vi "SDO_DRIVE_MODULE_OPEN.vi"(3 "Module Index":i32, 4 "RadiansPerCount":dbl=1.0, 5 "Drive PWM Channel":T2, 6 "DistancePerCount":dbl=1.0, 7 "Swerve PWM Channel":T2, 8 "Swerve B Channel":T1, 9 "Swerver A Channel":T1, 10 "Drive B Channel":T1, 11 "Drive A channel":T1) -> ()   [LabVIEW 2019]
uses:
  <vilib>/Rock Robotics/SystemInterfaces/DIO/FPGA_DIOChannel.ctl
  <vilib>/Rock Robotics/SystemInterfaces/DIO/FPGA_DIOPWMChannel.ctl
  <vilib>/Rock Robotics/WPI/MotorControl/WPI_MotorControlType.ctl
  <vilib>/Rock Robotics/WPI/PWM/WPI_PWMDeadband.ctl
  <vilib>/Rock Robotics/WPI/MotorControl/WPI_MotorControlDeviceRef.ctl
  <vilib>/Rock Robotics/SystemInterfaces/Encoder/FPGA_EncoderIdx.ctl
  <vilib>/Rock Robotics/SystemInterfaces/Counter/FPGA_CounterCtrSystemIndex.ctl
  <vilib>/Rock Robotics/WPI/Encoder/WPI_EncoderType.ctl
  <vilib>/Rock Robotics/WPI/Encoder/WPI_EncoderDevRef.ctl
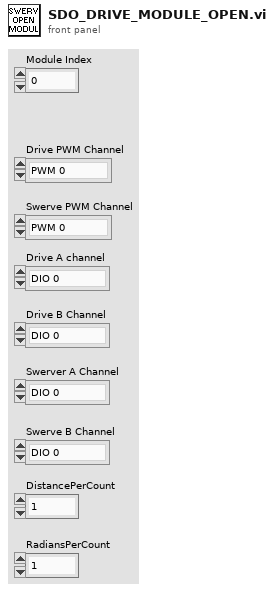
[diagram p1: front panel]
types:
  T1 = typedef "FPGA_DIOChannel.ctl" = enum8{"DIO 0", "DIO 1", "DIO 2", "DIO 3", "DIO 4", "DIO 5", "DIO 6", "DIO 7", "DIO 8", "DIO 9", "DIO MXP 0", "DIO MXP 1", "DIO MXP 2", "DIO MXP 3", "DIO MXP 4", "DIO MXP 5", "DIO MXP 6", "DIO MXP 7", "DIO MXP 8", "DIO MXP 9", "DIO MXP 10", "DIO MXP 11", "DIO MXP 12", "DIO MXP 13", "DIO MXP 14", "DIO MXP 15", "SPI Port CS1", "SPI Port CS2", "SPI Port CS3", "SPI Port MISO", "SPI Port MOSI", "Invalid"}
  T2 = typedef "FPGA_DIOPWMChannel.ctl" = enum8{"PWM 0", "PWM 1", "PWM 2", "PWM 3", "PWM 4", "PWM 5", "PWM 6", "PWM 7", "PWM 8", "PWM 9", "PWM MXP 0", "PWM MXP 1", "PWM MXP 2", "PWM MXP 3", "PWM MXP 4", "PWM MXP 5", "PWM MXP 6", "PWM MXP 7", "PWM MXP 8", "PWM MXP 9", "Invalid"}
  T3 = typedef "WPI_EncoderDevRef.ctl" = cluster{"DevStatus":errorcluster, "EncoderIndex":T4, "CounterIndex":T5, "DistancePerCount":dbl, "Decoding Type":T6}
  T4 = typedef "FPGA_EncoderIdx.ctl" = enum8{"Enc 0", "Enc 1", "Enc 2", "Enc 3", "Enc 4", "Enc 5", "Enc 6", "Enc 7", "Invalid"}
  T5 = typedef "FPGA_CounterCtrSystemIndex.ctl" = enum8{"Ctr 0", "Ctr 1", "Ctr 2", "Ctr 3", "Ctr 4", "Ctr 5", "Ctr 6", "Ctr 7", "Invalid"}
  T6 = typedef "WPI_EncoderType.ctl" = enum16{"1x", "2x", "4x"}
  T7 = typedef "WPI_MotorControlDeviceRef.ctl" = cluster{"DeviceStatus":errorcluster, "Type":T8, "PWM":cluster{"PWM Channel":T2, "DeadBand":T9}, "CAN":cluster{"Device Number":u8, "SetOutput VI Ref":variant, "GetOutput VI Ref":variant, "Enable VI Ref":variant, "Disable VI Ref":variant, "Data":variant}, "Invert":bool, "DIO PWM":cluster{"PWM \"Enable\" Channel":T2, "DIOChannel":T1, "PWM Rate":dbl}}
  T8 = typedef "WPI_MotorControlType.ctl" = enum16{"PWM", "CAN", "DIO PWM"}
  T9 = typedef "WPI_PWMDeadband.ctl" = cluster{"Name":string, "maxPositivePwm":i32, "minPositivePwm":i32, "centerPwm":i32, "maxNegativePwm":i32, "minNegativePwm":i32, "angularRange":u16}
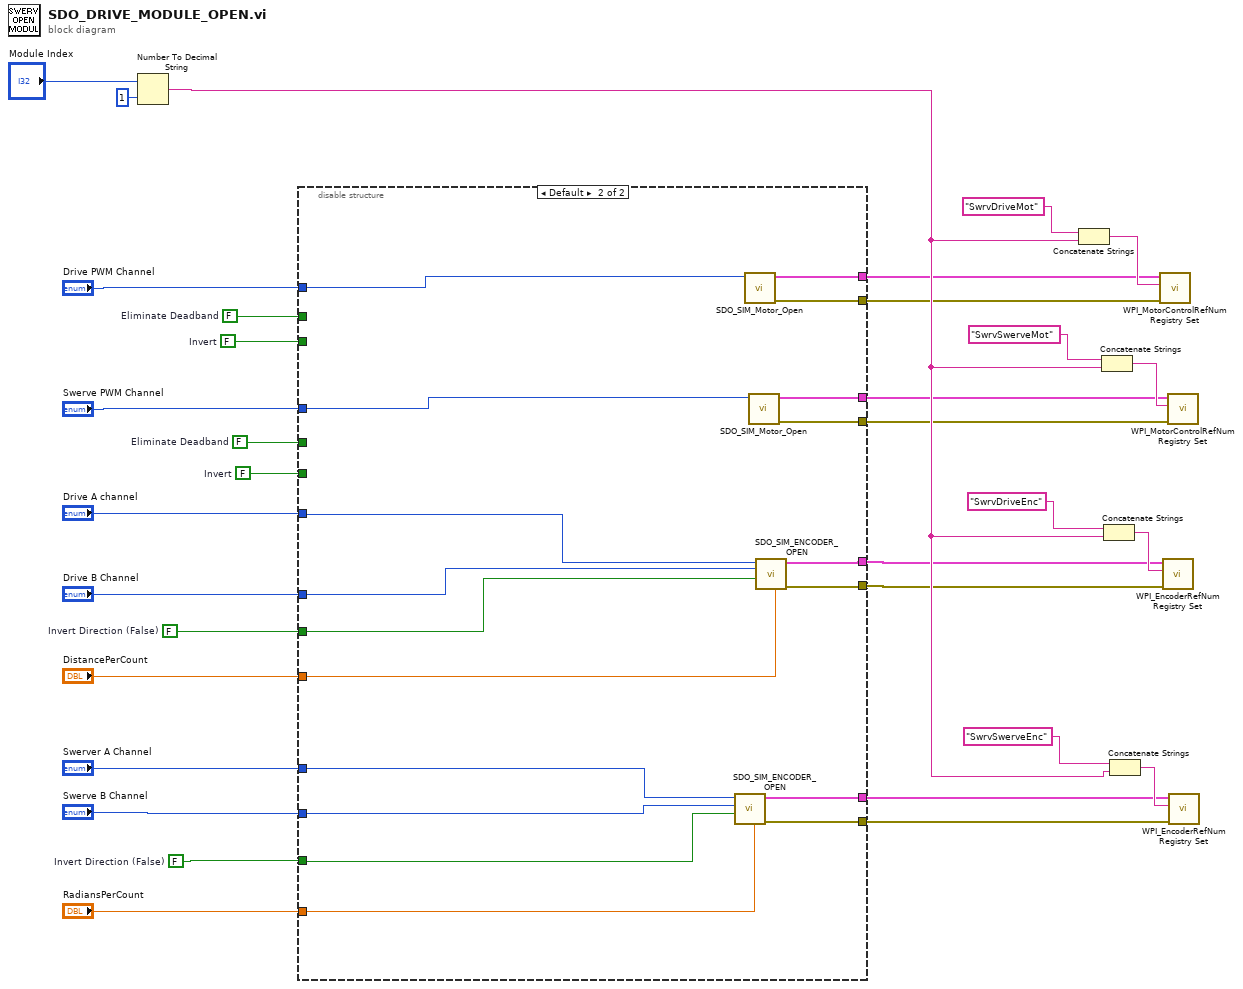
[diagram p0: block diagram]
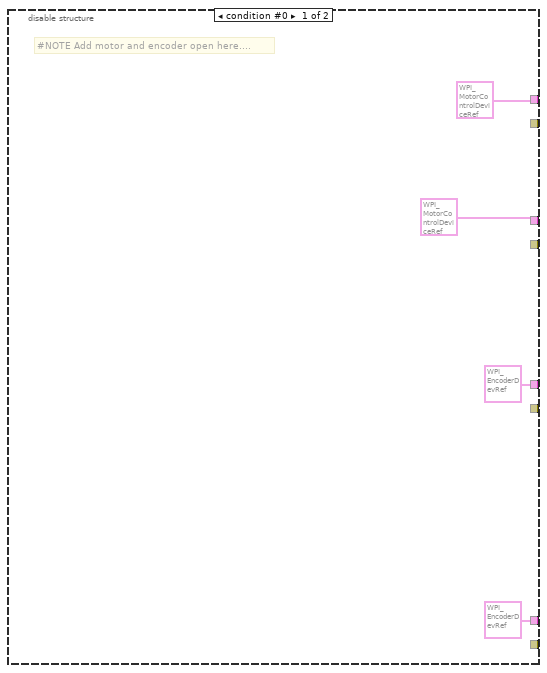
[diagram p2: hidden frame]
diagram:
  w2 = FALSE  # Eliminate Deadband
  w1 = FALSE  # Invert
  w4 = FALSE  # Invert
  w3 = FALSE  # Eliminate Deadband
  w5 = FALSE  # Invert Direction (False)
  w6 = FALSE  # Invert Direction (False)
  n1 = Number To Decimal String(number="Module Index", width (-)=i16 1) -> (decimal integer string=w15:string)
  n2 = disable-structure shown="Default" {
    disable-tunnel: "Swerve B Channel" -> [_ w47]
    disable-tunnel: "Swerver A Channel" -> [_ w46]
    disable-tunnel: "RadiansPerCount" -> [_ w49]
    disable-tunnel: "Drive B Channel" -> [_ w52]
    disable-tunnel: "Drive A channel" -> [_ w53]
    disable-tunnel: "DistancePerCount" -> [_ w50]
    disable-tunnel: "Swerve PWM Channel" -> [_ w42]
    disable-tunnel: "Drive PWM Channel" -> [_ w43]
    disable-tunnel: [_ w38] -> w14
    disable-tunnel: [T7 {"DeviceStatus"={"status"=FALSE, "code"=0, "source"=""}, "Type"=enum."PWM", "PWM"={"PWM Channel"=enum."Invalid", "DeadBand"={"Name"="", "maxPositivePwm"=0, "minPositivePwm"=0, "centerPwm"=0, "maxNegativePwm"=0, "minNegativePwm"=0, "angularRange"=0}}, "CAN"={"Device Number"=0, "SetOutput VI Ref"=variant, "GetOutput VI Ref"=variant, "Enable VI Ref"=variant, "Disable VI Ref"=variant, "Data"=variant}, "Invert"=FALSE, "DIO PWM"={"PWM \"Enable\" Channel"=enum."Invalid", "DIOChannel"=enum."Invalid", "PWM Rate"=0.0}} ("Motor Device Reference") w39] -> w13
    disable-tunnel: [_ w40] -> w12
    disable-tunnel: [T7 {"DeviceStatus"={"status"=FALSE, "code"=0, "source"=""}, "Type"=enum."PWM", "PWM"={"PWM Channel"=enum."Invalid", "DeadBand"={"Name"="", "maxPositivePwm"=0, "minPositivePwm"=0, "centerPwm"=0, "maxNegativePwm"=0, "minNegativePwm"=0, "angularRange"=0}}, "CAN"={"Device Number"=0, "SetOutput VI Ref"=variant, "GetOutput VI Ref"=variant, "Enable VI Ref"=variant, "Disable VI Ref"=variant, "Data"=variant}, "Invert"=FALSE, "DIO PWM"={"PWM \"Enable\" Channel"=enum."Invalid", "DIOChannel"=enum."Invalid", "PWM Rate"=0.0}} ("Motor Device Reference") w41] -> w11
    disable-tunnel: [_ w54] -> w10
    disable-tunnel: [T3 {"DevStatus"={"status"=FALSE, "code"=0, "source"=""}, "EncoderIndex"=enum."Invalid", "CounterIndex"=enum."Invalid", "DistancePerCount"=1.0, "Decoding Type"=enum."4x"} ("SwerveDriveEnc") w55] -> w9
    disable-tunnel: [_ w44] -> w8
    disable-tunnel: [T3 {"DevStatus"={"status"=FALSE, "code"=0, "source"=""}, "EncoderIndex"=enum."Invalid", "CounterIndex"=enum."Invalid", "DistancePerCount"=1.0, "Decoding Type"=enum."4x"} ("SwerveDriveEnc") w45] -> w7
    disable-tunnel: w6 -> [_ w48]
    disable-tunnel: w5 -> [_ w51]
    disable-tunnel: w4 -> [_ _]
    disable-tunnel: w3 -> [_ _]
    disable-tunnel: w2 -> [_ _]
    disable-tunnel: w1 -> [_ _]
    frame condition #0 {
      # "#NOTE Add motor and encoder open here...."
    }
    frame condition #1 (active) {
      n3 = call "SDO_SIM_ENCODER_OPEN.vi"("DistancePerCount"=w49, "Invert"=w48, "DIO Channel B"=w47, "DIO Channel  A"=w46) -> ("error out"=w44:errorcluster, "SwerveDriveEnc"=w45:T3)  [unwired: 6 in]
      n4 = call "SDO_SIM_Motor_Open.vi"("PWM Channel"=w43) -> ("error out"=w40:errorcluster, "Motor Device Reference"=w41:T7)  [unwired: 9 in]
      n5 = call "SDO_SIM_Motor_Open.vi"("PWM Channel"=w42) -> ("error out"=w38:errorcluster, "Motor Device Reference"=w39:T7)  [unwired: 9 in]
      n6 = call "SDO_SIM_ENCODER_OPEN.vi"("DistancePerCount"=w50, "Invert"=w51, "DIO Channel B"=w52, "DIO Channel  A"=w53) -> ("error out"=w54:errorcluster, "SwerveDriveEnc"=w55:T3)  [unwired: 6 in]
    }
  }
  n7 = Concatenate Strings("SwrvDriveMot" ("refnum name"), w15) -> (w16:string)
  n8 = Concatenate Strings("SwrvSwerveMot" ("refnum name"), w15) -> (w17:string)
  n9 = Concatenate Strings("SwrvDriveEnc" ("refnum name"), w15) -> (w18:string)
  n10 = Concatenate Strings("SwrvSwerveEnc" ("refnum name"), w15) -> (w19:string)
  n11 = call <vilib>:"WPI_MotorControlRefNum Registry Set.vi"("error in (no error)"=w12, "refnum name"=w16, "MotorControlDevRef"=w11) -> ()  [unwired: 7 in, 2 out]
  n12 = call <vilib>:"WPI_EncoderRefNum Registry Set.vi"("error in (no error)"=w10, "refnum name"=w18, "EncoderDevRef"=w9) -> ()  [unwired: 7 in, 2 out]
  n13 = call <vilib>:"WPI_MotorControlRefNum Registry Set.vi"("error in (no error)"=w14, "refnum name"=w17, "MotorControlDevRef"=w13) -> ()  [unwired: 7 in, 2 out]
  n14 = call <vilib>:"WPI_EncoderRefNum Registry Set.vi"("error in (no error)"=w8, "refnum name"=w19, "EncoderDevRef"=w7) -> ()  [unwired: 7 in, 2 out]
